vi "CSE - Link Error to Source Script.vi"(7 "get script source (T)":bool=TRUE, 8 "error in":errorcluster, 11 "CSE RefNum":T1) -> (0 "dup error in":errorcluster, 1 "statement info":T3 {"stmType" items=["expression", "jump", "source ref", "jump stub", "source stub"]}, 2 "Stm Index":i32, 3 "dup CSE RefNum":T1, 4 "this VI error":errorcluster, 5 "script":string, 6 "Error Message":string)   [LabVIEW 2021]
doc: "This VI returns information on the statement of a parsed script where either a parsing error or a runtime error occurred. This information links the invalid statement in the parsed script to the script source. It also provides additional information reflecting the statement's attributes used for execution, debugging, and messaging. Refer to the VI help for more details.\n\n::: CalcExpress Toolkit :::\nCopyright (c) 2000-2026 Konstantin Shifershteyn. All rights reserved."
uses:
  CSE Instance RefNum.ctl
  cetypes.llb/CalcExpress Instance RefNum.ctl
panel:
  # "Source Info"
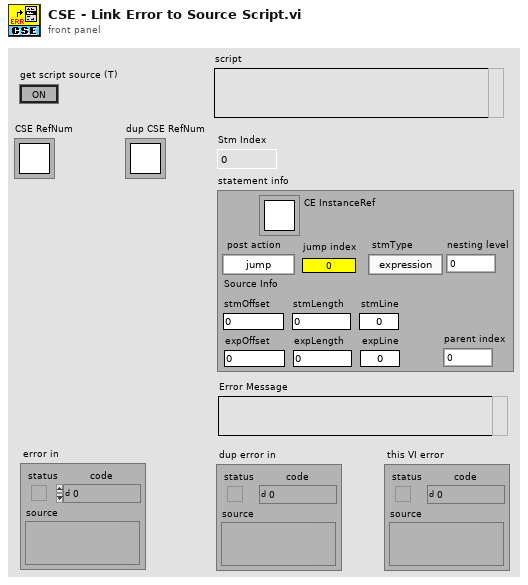
[diagram p1: front panel]
types:
  T1 = typedef "CSE Instance RefNum.ctl" = refnum<k1>
  T2 = typedef "CalcExpress Instance RefNum.ctl" = refnum<k1>
  T3 = cluster{"CE InstanceRef":T2, "post action":enum32{"jump", "jump if true", "jump if false", "stop"}, "jump index":i32, "stmType":i32, "nesting level":i32, "stmOffset":i32, "stmLength":i32, "stmLine ":i32, "expOffset":i32, "expLength":i32, "expLine":i32, "parent index":i32}
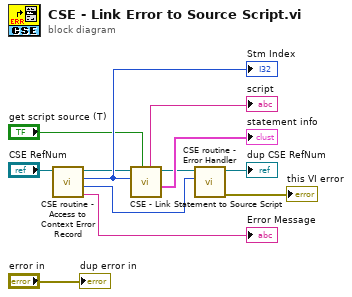
[diagram p0: block diagram]
diagram:
  n1 = call "CSE routine - Access to Context Error Record.vi"("CSE RefNum"="CSE RefNum") -> ("error message out"=→"Error Message":string, "error code out"=w6:i32, "Stm Index out"=w11:i32, "dup CSE RefNum"=w8:T1)  [unwired: 6 in, 1 out]
  "Stm Index" <- w11
  n2 = call "CSE - Link Statement to Source Script.vi"("get script source (T)"="get script source (T)", "Stm Index"=w11, "CSE RefNum"=w8) -> ("statement info"=→"statement info":T3, "dup CSE RefNum"=w7:T1, "script"=→"script":string)  [unwired: 3 in, 3 out]
  n3 = call "CSE routine - Error Handler.vi"("exec status"=w6, "CSE RefNum"=w7) -> ("error out"=→"this VI error":errorcluster, "dup CSE RefNum"=→"dup CSE RefNum":T1)  [unwired: 5 in, 1 out]
  "dup error in" <- "error in"
